vi "CIPC Universal FIFO.vi"() -> (3 "CIF_CIPC_Universal.lvclass":refnum<class "CIF_Iceoryx_Universal.lvclass">)   [LabVIEW 2021, in "CIF_Iceoryx_Universal.lvclass"]
uses:
  CIF_Iceoryx_Universal.lvclass
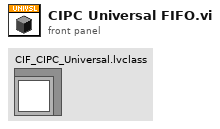
[diagram p1: front panel]
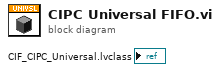
[diagram p0: block diagram]
diagram:
